vi "TCP Server Open Object Reference.vi"(8 "error in (no error)":errorcluster) -> (0 "error out":errorcluster, 3 "TCP Server Refnum":refnum<class "JKI TCP Server.lvclass">)   [LabVIEW 2020, in "JKI TCP Server.lvclass"]
uses:
  JKI TCP Server.lvclass
  JKI TCP Server.lvclass/JKI TCP Server.ctl
  _Data Structures/TCP Server Object Data Core Task Enum.ctl
  TCP Server Object Data Store.vi
panel:
  # "<VI NAME>\n\n<DESCRIPTION>\n\nCopyright (C) 2003 Jim Kring jim@jimkring.com\n\nPlease visit http://www.OpenG.org to learn about the\nOpen Source LabVIEW software movement.\n\nThis library is free software; you can redistribute it and/or\nmodify it under the terms of the GNU Lesser General Public\nLicense as published by the Free Software Foundation; either\nversion 2.1 of the License, or (at your option) any later version.\nThis library is distributed in the hope that it will be useful,\nbut WITHOUT ANY WARRANTY; without even the implied warranty of\nMERCHANTABILITY or FITNESS FOR A PARTICULAR PURPOSE. See the GNU\nLesser General Public License for more details.\nYou should have received a copy of the GNU Lesser General Public\nLicense along with this library; if not, write to the Free Software\nFoundation, Inc., 59 Temple Place, Suite 330, Boston, MA 02111-1307 USA"
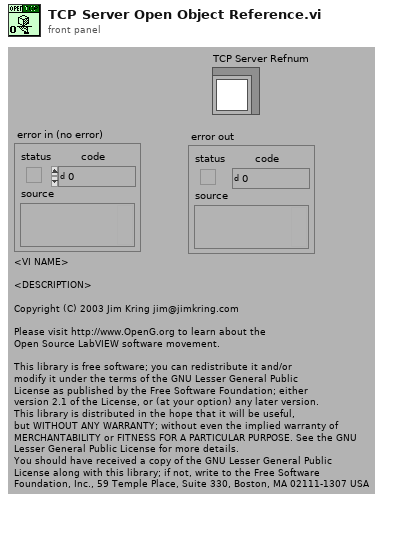
[diagram p1: front panel]
types:
  T1 = typedef "JKI TCP Server.lvclass/TCP Server Object Data Core Task Enum.ctl" = enum16{"read", "write", "init"}
  T2 = typedef "JKI TCP Server.lvclass/TCP Server Object RefNum.ctl" = refnum<k1>
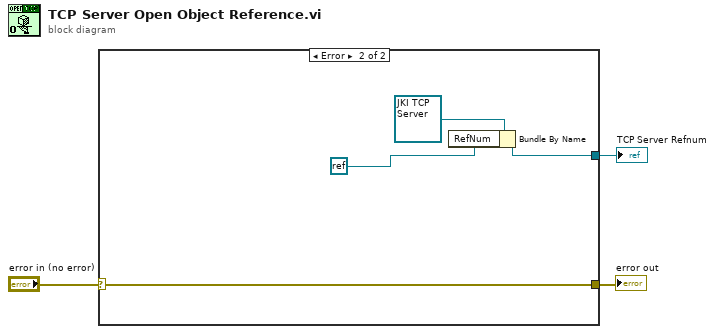
[diagram p0: block diagram]
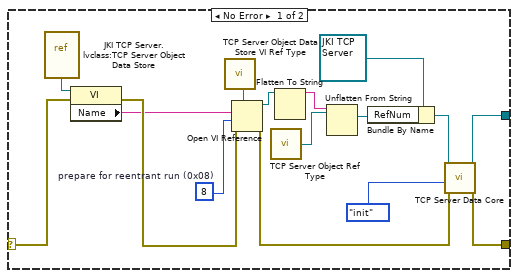
[diagram p2: hidden frame]
diagram:
  n1 = case shown="Error" "error in (no error)" {
    selector: "error in (no error)" -> [w10 w23]
    tunnel: [w13 w20] -> w3
    tunnel: [w12 w23] -> w2
    frame No Error {
      w19 = 8  # prepare for reentrant run (0x08)
      n2 = vi-ref "JKI TCP Server.lvclass:TCP Server Object Data Store.vi"() -> (w11:refnum<vi>)
      n3 = property class="VI"(reference=w11, error in=w10) -> (error out=w9:errorcluster, "Name"=w8:string)  [unwired: 1 out]
      n4 = call "TCP Server Object Data Store VI Ref Type.vi"() -> ("VI Refnum (Object Data Store.vi Type)"=w7:refnum<vi>)  [unwired: 5 in]
      n5 = Open VI Reference(type specifier VI Refnum (for type only)=w7, vi path=w8, options=w19, error in (no error)=w9) -> (vi reference=w18:refnum<vi>, error out=w14:errorcluster)  [unwired: 2 in]
      n6 = call "TCP Server Object Ref Type.vi"() -> ("Object RefNum Type"=w17:T2)  [unwired: 5 in]
      n7 = Flatten To String(anything=w18) -> (data string=w16:string)  [unwired: 3 in, 2 out]
      n8 = Unflatten From String(type=w17, binary string=w16) -> (value=w5:T2)  [unwired: 3 in, 2 out]
      n9 = Bundle By Name(cluster=refnum<class "JKI TCP Server.lvclass"> refnum ("TCP Server Refnum"), "RefNum"=w5) -> (w4:refnum<class "JKI TCP Server.lvclass">)
      n10 = call "TCP Server Data Core.vi"("error in (no error)"=w14, "task (read)"=TCP_Server_Object_Data_Core_Task_Enum."init", "Refnum"=w4) -> ("error out"=w12:errorcluster, "dup Refnum"=w13:refnum<class "JKI TCP Server.lvclass">)  [unwired: 6 in, 1 out]
    }
    frame Error {
      n11 = Bundle By Name(cluster=refnum<class "JKI TCP Server.lvclass"> refnum ("TCP Server Refnum"), "RefNum"=refnum<k0> refnum) -> (w20:refnum<class "JKI TCP Server.lvclass">)
    }
  }
  "error out" <- w2
  "TCP Server Refnum" <- w3
